vi "WriteAO.vi"(7 "GroveConnector":enum16{"A0", "A1", "A2"}(ring), 8 "error in (no error)":errorcluster, 9 "Duty Cycle %":sgl=0.091836736, 10 "Frequency Hz":sgl=0.001, 11 "Session in":refnum<class "Session.lvclass">) -> (0 "error out":errorcluster, 3 "Session out":refnum<class "Session.lvclass">)   [LabVIEW 2020]
doc: "Establishes communication with the instrument and optionally performs an instrument identification query and/or an instrument reset. It also places the instrument in a default state needed for other instrument driver operations. Therefore, call this VI before calling other instrument driver VIs for this instrument. Generally, you need to call the <b>Initialize</b> VI only once at the beginning of an application."
uses:
  CTI/Session/Session.lvclass
  CTI/GPIO Number.ctl
  CTI/CTI.lvlib
panel:
  # "Input"
  # "Output"
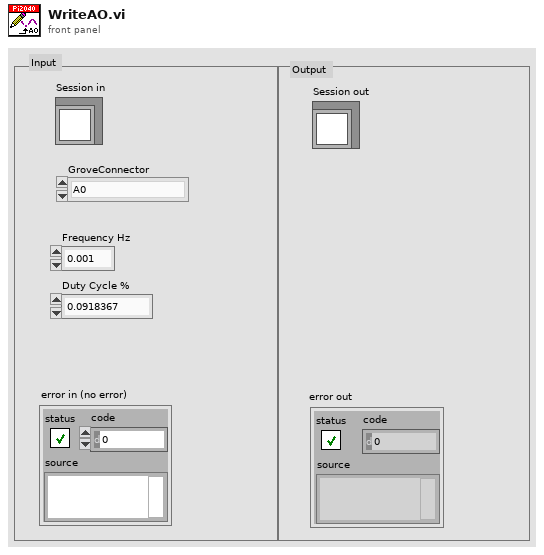
[diagram p1: front panel]
types:
  T1 = typedef "CTI.lvlib/GPIO Number.ctl" = i8
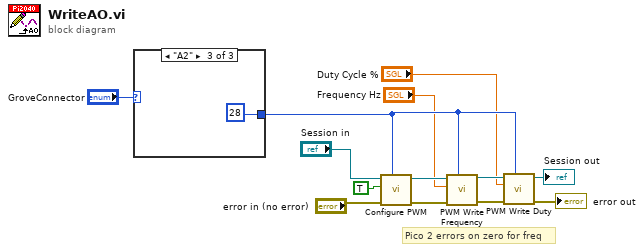
[diagram p0: block diagram]
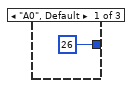
[diagram p2: hidden frame]
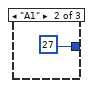
[diagram p3: hidden frame]
diagram:
  # "Pico 2 errors on zero for freq"
  n1 = case shown="\"A2\"" "GroveConnector" {
    tunnel: [T1 26 ("GPIO #") T1 27 ("GPIO #") T1 28 ("GPIO #")] -> w9
    frame "A0", Default {
    }
    frame "A1" {
    }
    frame "A2" {
    }
  }
  n2 = call "Configure PWM.vi"("GPIO #"=w9, "error in (no error)"="error in (no error)", "Enable (F)"=TRUE, "Session in"="Session in") -> ("error out"=w11:errorcluster, "Session out"=w10:refnum<class "Session.lvclass">)  [unwired: 6 in]
  n3 = call "PWM Write Frequency.vi"("GPIO #"=w9, "error in (no error)"=w11, "Frequency Hz"="Frequency Hz", "Session in"=w10) -> ("error out"=w5:errorcluster, "Session out"=w6:refnum<class "Session.lvclass">)  [unwired: 6 in]
  n4 = call "PWM Write Duty.vi"("GPIO #"=w9, "error in (no error)"=w5, "Duty % (0-1)"="Duty Cycle %", "Session in"=w6) -> ("error out"=→"error out":errorcluster, "Session out"=→"Session out":refnum<class "Session.lvclass">)  [unwired: 6 in]
